vi "!Test-Sgraph-system.vi"() -> ()   [LabVIEW 2020, in "Sgraph_lib_V1.lvlib"]
uses:
  Builds/Sgraph_lib_V1.lvlib
  <vilib>/Platform/TimedLoop/XDataNode/timing_clust.ctl
  <vilib>/Platform/TimedLoop/XDataNode/nitl_modes.ctl
  <vilib>/Platform/TimedLoop/XDataNode/wakeup.ctl
  Common/controls/Global-services.vi
  <vilib>/platform/TimedLoop/XDataNode/XDataNode.xnode
  <vilib>/Platform/TimedLoop/XDataNode/XDNodeRunTimeDep.lvlib
  Gserver/Gserver.lvclass
  HISW/HISW.lvclass
panel:
  in  "DBAL":bool
  in  "M Map":bool caption="Memory Map"
  out "HISW-queue":i32
  in  "OpenGraph":bool caption="Graph"
  out "HMI-error":bool
  out "Numeric":i32
  in  "Gserver":bool
  in  "FAMM":bool
  in  "HISW":bool
  in  "Stop DAQ":bool
  out "DAQ":picture
  in  "DAQ":bool
  # "Test Sgraph data historian test utility"
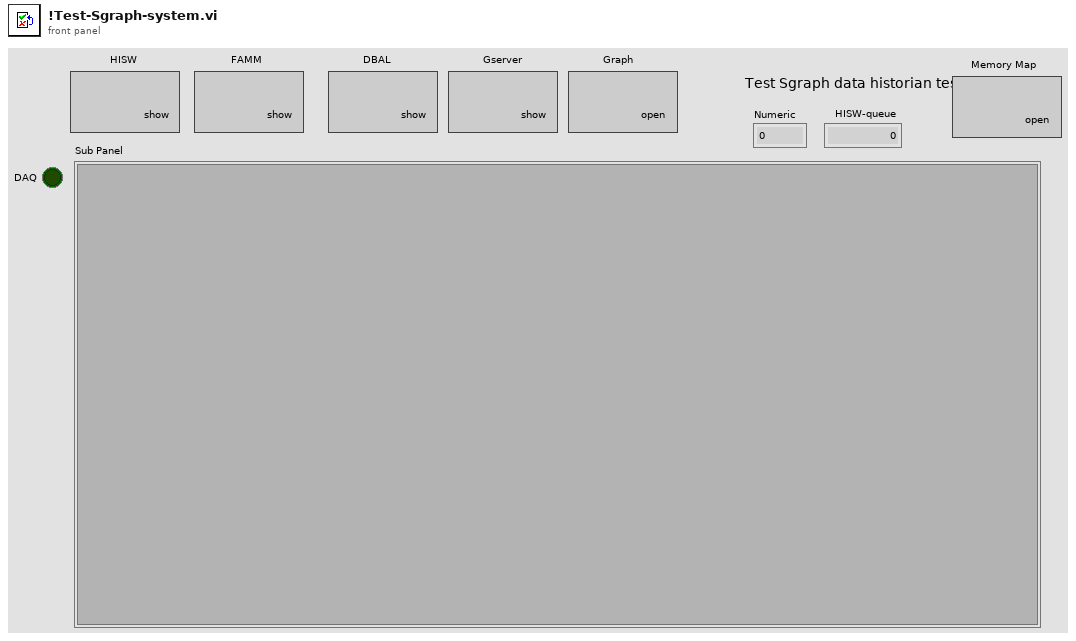
[diagram p1: front panel]
types:
  T1 = typedef "XDNodeRunTimeDep.lvlib/timing_clust.ctl" = cluster{"Expected End [f-1]":u64, "Actual End [f-1]":u64, "Finished Late? [f-1]":bool, "Expected End [i-1]":u64, "Actual End [i-1]":u64, "Finished Late? [i-1]":bool, "Expected Start [i]":u64, "Actual Start [i]":u64, "Expected Start [f]":u64, "Actual Start [f]":u64, "Source Name":string, "Structure Name":string, "Period":i64, "Deadline":i64, "Offset":i64, "Start":i64, "Priority":i32, "Timeout":i32, "Mode":T2, "Wakeup Reason":T3, "Error":errorcluster, "Source Type":string, "Secondary Source Type":string, "Global End Time":u64, "Global Start Time":u64, "Frame Duration":u64, "Iteration Duration":u64, "Assigned CPU":i32, "I/O Scan Engine Mode":u32}
  T2 = typedef "XDNodeRunTimeDep.lvlib/nitl_modes.ctl" = enum32{"No Change", "Process missed periods, maintain original phase", "Discard missed periods, maintain original phase", "Process missed periods, ignore original phase", "Discard missed periods, ignore original phase"}
  T3 = typedef "XDNodeRunTimeDep.lvlib/wakeup.ctl" = enum32{"Normal", "Aborted", "Asynchronous wakeup", "Timing source error", "Timed loop error", "Timeout"}
  T4 = typedef "typedef_PAQsample.ctl" = cluster{"Time Stamp":timestamp, "TAGs":string[], "status":u32[], "data":dbl[], "Source":string}
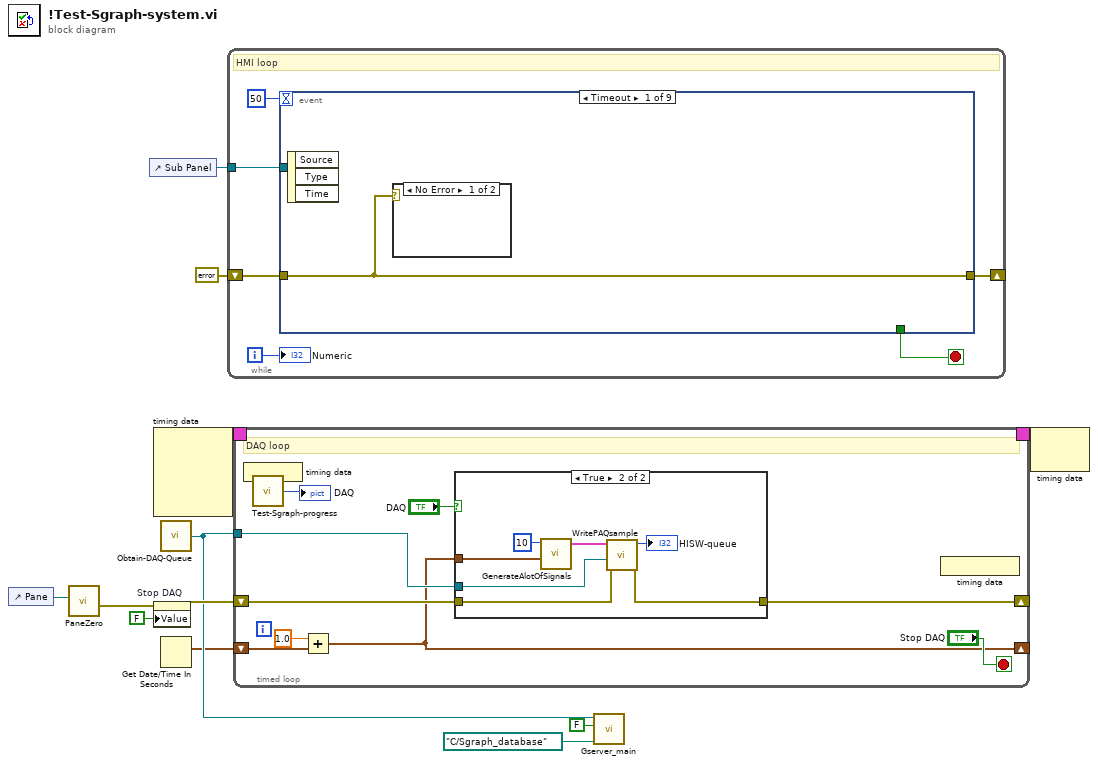
[diagram p0: block diagram]
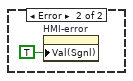
[diagram p3: hidden frame]
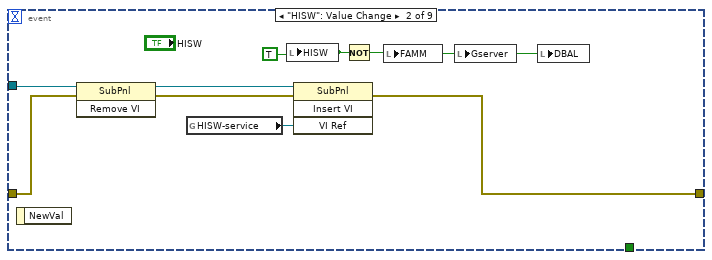
[diagram p4: hidden frame]
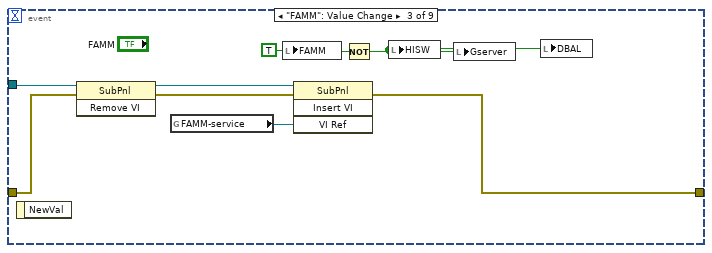
[diagram p5: hidden frame]
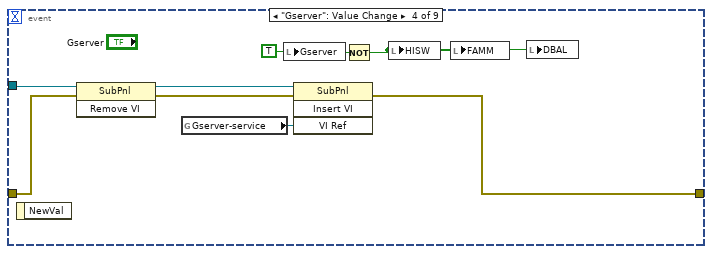
[diagram p6: hidden frame]
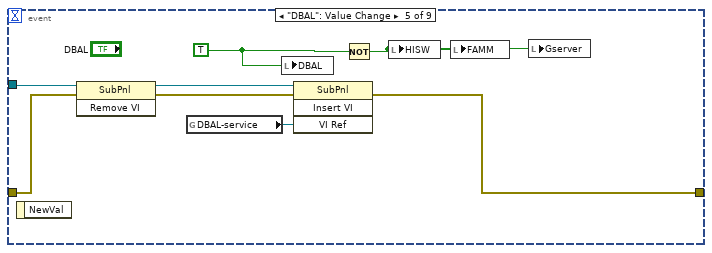
[diagram p7: hidden frame]
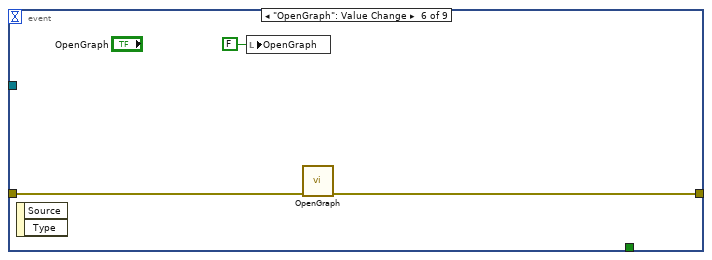
[diagram p8: hidden frame]
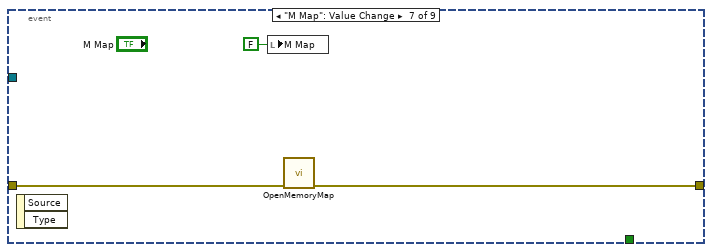
[diagram p9: hidden frame]
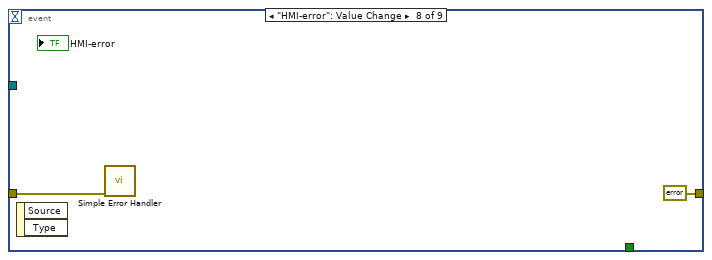
[diagram p10: hidden frame]
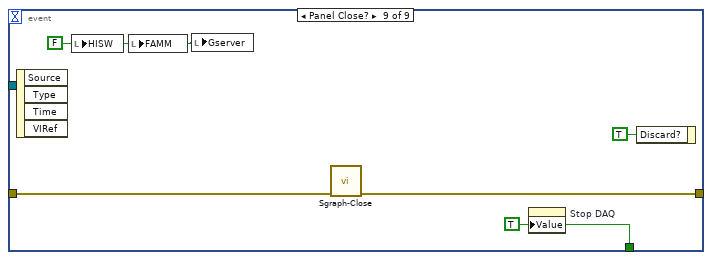
[diagram p11: hidden frame]
diagram:
  n1 = control-ref of="Pane"() -> (w5:refnum<vi>)
  n2 = call "PaneZero.vi"("Pane"=w5) -> ("error out"=w6:errorcluster)  [unwired: 10 in]
  n3 = control-ref of="Sub Panel"() -> (w8:refnum<vi>)
  n4 = node-c288() -> (w12:T1)  [unwired: 4 in]
  n5 = property on="Stop DAQ" class="Bool (strict)"(error in=w6, "Value"=FALSE ("Stop DAQ")) -> (error out=w9:errorcluster)  [unwired: 1 in, 1 out]
  n6 = call "Obtain-DAQ-Queue.vi"() -> ("DAQ-Queue"=w4:refnum<queue>)  [unwired: 7 in]
  n7 = Get Date/Time In Seconds() -> (seconds since 1Jan1904=w3:timestamp)
  n8 = while {
    tunnel: w8 -> [w17]
    shift-right: [w16] -> _
    shift-left: errorcluster {"status"=FALSE, "code"=0, "source"=""} ("error out") -> [w15]
    i -> [w13]
    stop <- w14 stop-if-true
    # "HMI loop"
    n9 = event shown="[0] Timeout" {
      selector: _ -> [_ _ _ _ _ _ _ _ _]
      dyn-events: _ -> [_ _ _ _ _ _ _ _ _]
      timeout: 50 -> [_ _ _ _ _ _ _ _ _]
      tunnel: [_ _ _ _ _ _ _ _ w64] -> w14
      tunnel: w17 -> [_ w27 w36 w44 w52 _ _ _ _]
      tunnel: [w19 w23 w32 w40 w48 w54 w58 errorcluster {"status"=FALSE, "code"=0, "source"=""} ("error out") w62] -> w16
      tunnel: w15 -> [w19 w22 w31 w39 w47 w53 w57 w59 w63]
      event Timeout {
        n10 = event-data() -> ()  [unwired: 1 in, 3 out]
        n11 = case shown="No Error" w19 {
          frame No Error {
          }
          frame Error {
            n12 = property on="HMI-error" class="Bool (strict)"("Val(Sgnl)"=TRUE ("Value (Signaling)")) -> ()  [unwired: 2 in, 2 out]
          }
        }
      }
      event "HISW": Value Change {
        w28 = TRUE ("HISW")
        n13 = event-data() -> ()  [unwired: 1 in, 1 out]
        n14 = invoke class="SubPnl" method="Remove VI"(reference=w27, error in=w22) -> (reference out=w26:refnum<vi>, error out=w24:errorcluster)  [unwired: 1 in, 1 out]
        n15 = global read "Global-services.vi" "HISW-service"() -> (w25:refnum<vi>)
        n16 = local write "HISW"(w28) -> ()
        n17 = invoke class="SubPnl" method="Insert VI"(reference=w26, error in=w24, "VI Ref"=w25) -> (error out=w23:errorcluster)  [unwired: 1 in, 3 out]
        n18 = Not(x=w28) -> (.not. x?=w21:bool)
        n19 = local write "FAMM"(w21) -> ()
        n20 = local write "Gserver"(w21) -> ()
        n21 = local write "DBAL"(w21) -> ()
      }
      event "FAMM": Value Change {
        w30 = TRUE ("HISW")
        n22 = event-data() -> ()  [unwired: 1 in, 1 out]
        n23 = invoke class="SubPnl" method="Remove VI"(reference=w36, error in=w31) -> (reference out=w35:refnum<vi>, error out=w33:errorcluster)  [unwired: 1 in, 1 out]
        n24 = global read "Global-services.vi" "FAMM-service"() -> (w34:refnum<vi>)
        n25 = local write "FAMM"(w30) -> ()
        n26 = invoke class="SubPnl" method="Insert VI"(reference=w35, error in=w33, "VI Ref"=w34) -> (error out=w32:errorcluster)  [unwired: 1 in, 3 out]
        n27 = Not(x=w30) -> (.not. x?=w29:bool)
        n28 = local write "HISW"(w29) -> ()
        n29 = local write "Gserver"(w29) -> ()
        n30 = local write "DBAL"(w29) -> ()
      }
      event "Gserver": Value Change {
        w38 = TRUE ("HISW")
        n31 = event-data() -> ()  [unwired: 1 in, 1 out]
        n32 = invoke class="SubPnl" method="Remove VI"(reference=w44, error in=w39) -> (reference out=w43:refnum<vi>, error out=w41:errorcluster)  [unwired: 1 in, 1 out]
        n33 = global read "Global-services.vi" "Gserver-service"() -> (w42:refnum<vi>)
        n34 = local write "Gserver"(w38) -> ()
        n35 = invoke class="SubPnl" method="Insert VI"(reference=w43, error in=w41, "VI Ref"=w42) -> (error out=w40:errorcluster)  [unwired: 1 in, 3 out]
        n36 = Not(x=w38) -> (.not. x?=w37:bool)
        n37 = local write "HISW"(w37) -> ()
        n38 = local write "FAMM"(w37) -> ()
        n39 = local write "DBAL"(w37) -> ()
      }
      event "DBAL": Value Change {
        w46 = TRUE ("HISW")
        n40 = event-data() -> ()  [unwired: 1 in, 1 out]
        n41 = invoke class="SubPnl" method="Remove VI"(reference=w52, error in=w47) -> (reference out=w51:refnum<vi>, error out=w49:errorcluster)  [unwired: 1 in, 1 out]
        n42 = global read "Global-services.vi" "DBAL-service"() -> (w50:refnum<vi>)
        n43 = local write "DBAL"(w46) -> ()
        n44 = invoke class="SubPnl" method="Insert VI"(reference=w51, error in=w49, "VI Ref"=w50) -> (error out=w48:errorcluster)  [unwired: 1 in, 3 out]
        n45 = Not(x=w46) -> (.not. x?=w45:bool)
        n46 = local write "HISW"(w45) -> ()
        n47 = local write "FAMM"(w45) -> ()
        n48 = local write "Gserver"(w45) -> ()
      }
      event "OpenGraph": Value Change {
        n49 = event-data() -> ()  [unwired: 1 in, 2 out]
        n50 = local write "OpenGraph"(FALSE ("OpenGraph")) -> ()
        n51 = call "OpenGraph.vi"("error in (no error)"=w53) -> ("Error out"=w54:errorcluster)  [unwired: 10 in]
      }
      event "M Map": Value Change {
        n52 = event-data() -> ()  [unwired: 1 in, 2 out]
        n53 = local write "M Map"(FALSE ("M Map")) -> ()
        n54 = call "OpenMemoryMap.vi"("error in (no error)"=w57) -> ("Error out"=w58:errorcluster)  [unwired: 10 in]
      }
      event "HMI-error": Value Change {
        n55 = event-data() -> ()  [unwired: 1 in, 2 out]
        n56 = call <vilib>:"Simple Error Handler.vi"("error in (no error)"=w59) -> ()  [unwired: 4 in, 5 out]
      }
      event Panel Close? {
        w61 = FALSE ("HISW")
        w64 = TRUE ("Stop DAQ")
        n57 = event-data() -> ()  [unwired: 1 in, 4 out]
        n58 = local write "HISW"(w61) -> ()
        n59 = local write "FAMM"(w61) -> ()
        n60 = local write "Gserver"(w61) -> ()
        n61 = call "Sgraph-Close.vi"("error in (no error)"=w63) -> ("error out"=w62:errorcluster)  [unwired: 10 in]
        n62 = property on="Stop DAQ" class="Bool (strict)"("Value"=w64) -> ()  [unwired: 2 in, 2 out]
        n63 = event-data("Discard?"=TRUE) -> ()  [unwired: 1 in, 1 out]
      }
    }
    "Numeric" <- w13
  }
  n64 = timed-loop {
    timing: w12 -> [_]
    timing-out: [_] -> w11
    shift-right: [w70] -> _
    shift-left: w9 -> [w71]
    tunnel: w4 -> [w69]
    shift-right: [w66] -> _
    shift-left: w3 -> [w68]
    stop <- "Stop DAQ" stop-if-true
    # "DAQ loop"
    n65 = node-c288() -> ()  [unwired: 1 in]
    n66 = call "Test-Sgraph-progress.vi"() -> ("37x37"=→"DAQ":picture)  [unwired: 7 in]
    n67 = Add(x=1.0, y=w68) -> (x+y=w66:timestamp)
    n68 = case shown="True" "DAQ" {
      tunnel: w71 -> [w75 w80]
      tunnel: [w75 w79] -> w70
      tunnel: w69 -> [_ w78]
      tunnel: w66 -> [_ w76]
      frame False {
      }
      frame True {
        n69 = call "GenerateAlotOfSignals.vi"("Time"=w76, "Channels"=10) -> ("DAQ"=w81:T4)  [unwired: 9 in]
        n70 = call "WritePAQsample.vi"("error in (no error)"=w80, "DAQ-Queue"=w78, "PAQ IN"=w81) -> ("error out"=w79:errorcluster, "# elements in queue"=→"HISW-queue":i32)  [unwired: 7 in]
      }
    }
    n71 = node-c288() -> ()  [unwired: 1 out]
  }
  n72 = call "Gserver_main.vi"("Database location"=path "C:/Sgraph_database", "debug"=FALSE, "DAQ-Queue"=w4) -> ()  [unwired: 9 in]
  n73 = node-c288(w11) -> ()  [unwired: 1 out]
